vi "Store Measuement Config.vi"(8 "error in (no error)":errorcluster, 10 "Measurement Setup Controller.lvlib:Measurement Data.lvclass":refnum<class "Measurement Data.lvclass">, 11 "Measurement Setup in":refnum<class "Measurement Setup.lvclass">) -> (0 "error out":errorcluster, 3 "Measurement Setup out":refnum<class "Measurement Setup.lvclass">)   [LabVIEW 2017, in "Measurement Setup Controller.lvlib" / "Measurement Setup.lvclass"]
uses:
  Measurement Setup.lvclass
  C:/Program Files (x86)/National Instruments/LabVIEW 2017/user.lib/Common Components/Controller/Controller.lvclass
  C:/Program Files (x86)/National Instruments/LabVIEW 2017/vi.lib/ActorFramework/Actor/Actor.lvclass
  Measurement Data/Measurement Data.lvclass
  Measurement Data/Measurement Data.lvclass/Measurement Data.ctl
  <userlib>/Common Components/Measurement Actor/Measurement.lvclass/Measurement.ctl
  Measurement Setup.lvclass/Measurement Setup.ctl
  <vilib>/ActorFramework/Actor/Actor.lvclass/Actor.ctl
  <vilib>/ActorFramework/Message Enqueuer/Message Enqueuer.lvclass/Message Enqueuer.ctl
  <vilib>/ActorFramework/Message Enqueuer/Init from Existing Queue.vi
  <vilib>/ActorFramework/Message Enqueuer/Enqueue.vi
  <vilib>/ActorFramework/Stop Msg/Stop Msg.lvclass
  C:/Program Files (x86)/National Instruments/LabVIEW 2017/vi.lib/ActorFramework/Message/Message.lvclass
  <vilib>/ActorFramework/Message Priority Queue/Priority Enqueue.vi
  <vilib>/ActorFramework/Message Enqueuer/Message Enqueuer.lvclass
  <userlib>/Common Components/Measurement Actor/Configuration/Step Configuration.lvclass
  <userlib>/Common Components/Hardware/Hardware.lvclass
  <vilib>/ActorFramework/Actor/Actor.lvclass
  <userlib>/Common Components/Controller/Controller.lvclass
  <userlib>/Common Components/Measurement Actor/Measurement.lvclass
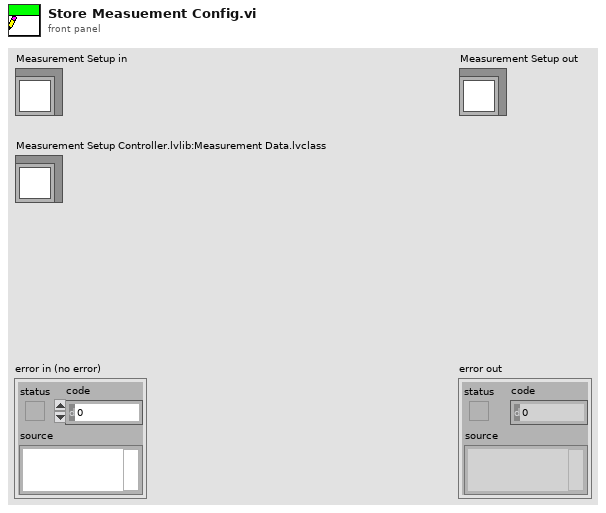
[diagram p1: front panel]
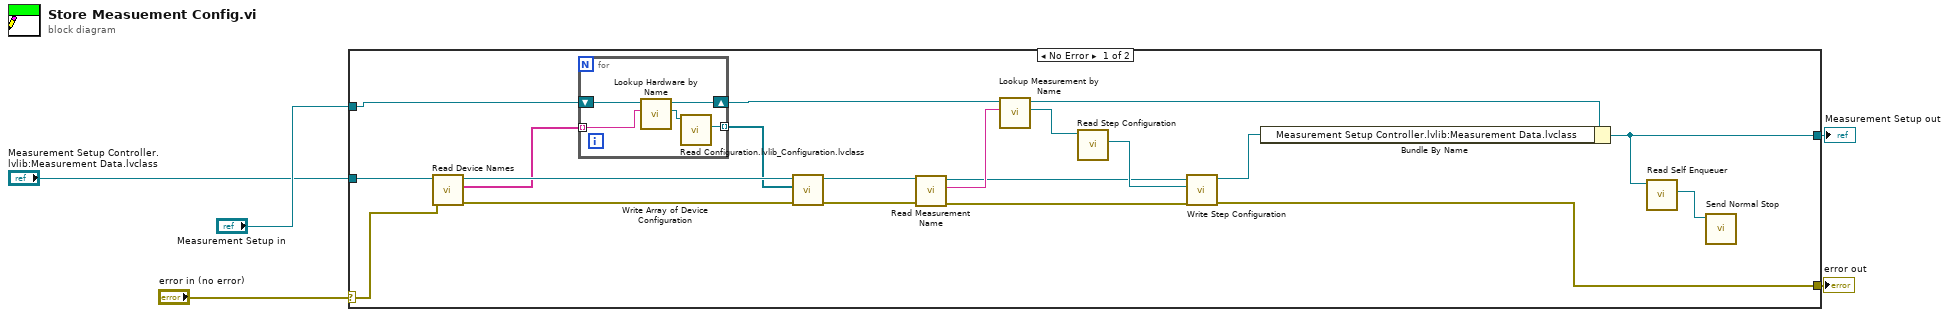
[diagram p0: block diagram]
diagram:
  n1 = case shown="No Error" "error in (no error)" {
    selector: "error in (no error)" -> [w13 w31]
    tunnel: [w11 w31] -> w4
    tunnel: [w25 w32] -> w2
    tunnel: "Measurement Setup in" -> [w16 w32]
    tunnel: "Measurement Setup Controller.lvlib:Measurement Data.lvclass" -> [w22 _]
    frame No Error {
      n2 = call "Read Device Names.vi"("error in (no error)"=w13, "Measurement Data in"=w22) -> ("error out"=w12:errorcluster, "Device Names"=w18:string[], "Measurement Data out"=w21:refnum<class "Measurement Data.lvclass">)  [unwired: 7 in]
      n3 = for {
        tunnel: w18 -> [w30] mode=indexing
        tunnel: [w27] -> w17 mode=indexing
        shift-right: [w26] -> w15
        shift-left: w16 -> [w29]
        n4 = call <userlib>:"Lookup Hardware by Name.vi"("Device Name"=w30, "Controller in"=w29) -> ("Hardware.lvclass"=w28:refnum<class "Hardware.lvclass">, "Controller out"=w26:refnum<class "Measurement Setup.lvclass">)  [unwired: 7 in, 1 out]
        n5 = call-dynamic "Read Configuration.lvlib_Configuration.lvclass.vi"("Hardware in"=w28) -> ("Hardware.lvlib:HW Configuration.lvclass"=w27:refnum<class "HW Configuration.lvclass">)  [unwired: 8 in, 2 out]
      }
      n6 = call "Write Array of Device Configuration.vi"("error in (no error)"=w12, "Array of Device Configuration"=w17, "Measurement Data in"=w21) -> ("error out"=w7:errorcluster, "Measurement Data out"=w10:refnum<class "Measurement Data.lvclass">)  [unwired: 7 in]
      n7 = call "Read Measurement Name.vi"("error in (no error)"=w7, "Measurement Data in"=w10) -> ("error out"=w6:errorcluster, "Measurement Name"=w9:string, "Measurement Data out"=w8:refnum<class "Measurement Data.lvclass">)  [unwired: 7 in]
      n8 = call <userlib>:"Lookup Measurement by Name.vi"("Measurement Name"=w9, "Controller in"=w15) -> ("Measurement.lvclass"=w20:refnum<class "Measurement.lvclass">, "Controller out"=w14:refnum<class "Measurement Setup.lvclass">)  [unwired: 6 in, 2 out]
      n9 = call <userlib>:"Read Step Configuration.vi"("Measurement in"=w20) -> ("Measurement Actor.lvlib:Step Configuration.lvclass"=w19:refnum<class "Step Configuration.lvclass">)  [unwired: 8 in, 2 out]
      n10 = call "Write Step Configuration.vi"("error in (no error)"=w6, "Measurement Actor.lvlib:Step Configuration.lvclass"=w19, "Measurement Data in"=w8) -> ("error out"=w11:errorcluster, "Measurement Data out"=w23:refnum<class "Measurement Data.lvclass">)  [unwired: 7 in]
      n11 = Bundle By Name(cluster=w14, "Measurement Setup Controller.lvlib:Measurement Data.lvclass"=w23) -> (w25:refnum<class "Measurement Setup.lvclass">)
      n12 = call <vilib>:"Read Self Enqueuer.vi"("Actor"=w25) -> ("Self Enqueuer"=w24:refnum<class "Message Enqueuer.lvclass">)  [unwired: 10 in]
      n13 = call <vilib>:"Send Normal Stop.vi"("Message Enqueuer"=w24) -> ()  [unwired: 10 in, 1 out]
    }
    frame Error {
    }
  }
  "error out" <- w4
  "Measurement Setup out" <- w2
